vi "Test Search-Split String.vi"(8 "error in (no error)":errorcluster) -> (0 "error out":errorcluster, 3 "Pass?":bool)   [LabVIEW 2020]
uses:
  G-Unicode/Types/UTF-8 String/UTF-8 String.lvclass/UTF-8 String.ctl
  9ff3dfa9-f8ba-4427-ad5f-a2fde7b6c77a.vi
  850149eb-9a48-45f9-aca9-3728815fdd3d.vi
  d33158b6-7e12-4a86-8fbe-645f2238ccec.vi
  2fcd0a92-766f-4ab9-bfdc-e2927028f498.vi
  451e0aa1-621d-4b4c-868c-abfc6350e238.vi
  77c8659a-ed0f-4c8d-a4b1-7b3f6f0d4640.vi
  G-Unicode/Private/Conversion/String as Encoded String.vi
  G-Unicode/Private/Conversion/Polymorphic VIs/String as Encoded String (LabVIEW String).vi
  G-Unicode/Private/Library/gu_search_split_string.vi
  850149eb-9a48-45f9-aca9-3728815fdd3d.vi/3a31b270-3bb6-4c58-a256-c5fcc2c98f09.vi
  850149eb-9a48-45f9-aca9-3728815fdd3d.vi/0ec5df2d-ef9b-4f84-a6a8-ffcedd45c4dc.vi
  d33158b6-7e12-4a86-8fbe-645f2238ccec.vi/3a31b270-3bb6-4c58-a256-c5fcc2c98f09.vi
  d33158b6-7e12-4a86-8fbe-645f2238ccec.vi/0ec5df2d-ef9b-4f84-a6a8-ffcedd45c4dc.vi
  451e0aa1-621d-4b4c-868c-abfc6350e238.vi/3a31b270-3bb6-4c58-a256-c5fcc2c98f09.vi
  451e0aa1-621d-4b4c-868c-abfc6350e238.vi/0ec5df2d-ef9b-4f84-a6a8-ffcedd45c4dc.vi
  77c8659a-ed0f-4c8d-a4b1-7b3f6f0d4640.vi/3a31b270-3bb6-4c58-a256-c5fcc2c98f09.vi
  77c8659a-ed0f-4c8d-a4b1-7b3f6f0d4640.vi/0ec5df2d-ef9b-4f84-a6a8-ffcedd45c4dc.vi
  G-Unicode/Private/Conversion/Text to UTF-8.vi
  G-Unicode/Private/Conversion/Polymorphic VIs/Text to UTF-8 (LabVIEW String).vi
  G-Unicode/Private/Memory/Copy String.vi
  G-Unicode/Private/Library/Result To Error.vi
  G-Unicode/Private/Conversion/Text as Encoded String.vi
  G-Unicode/Private/Conversion/Polymorphic VIs/Text as Encoded String (LabVIEW String).vi
  G-Unicode/Private/Conversion/Polymorphic VIs/Text as Encoded String (UTF-8 String).vi
  G-Unicode/Private/Memory/Copy String.vi/4d47babd-4a2d-4eb7-b91b-7e707d692665.vi
  G-Unicode/Private/Library/gu_free.vi
  G-Unicode/Types/UTF-8 String/Read Encoded UTF-8 String.vi
  <vilib>/Utility/error.llb/Error Cluster From Error Code.vi
  G-Unicode/Types/UTF-8 String/UTF-8 String.lvclass
  f040e557-eb9e-442d-a968-7fe909837c60.vi
  G-Unicode/Unicode/Controls/String Encoding.ctl
  G-Unicode/G-Unicode.lvlib
  6d55fd50-21d3-485a-937b-971210f7077f.vi
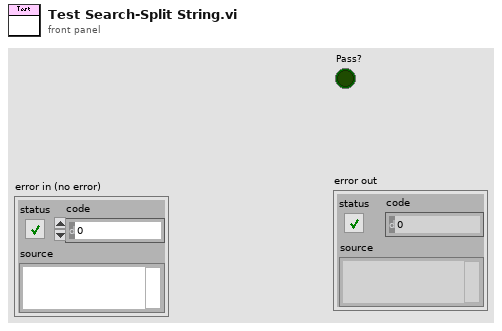
[diagram p1: front panel]
types:
  T1 = typedef "G-Unicode.lvlib/String Encoding.ctl" = enum16{"ANSI", "UTF-8", "UTF-16LE", "UTF-16BE", "Unknown"}
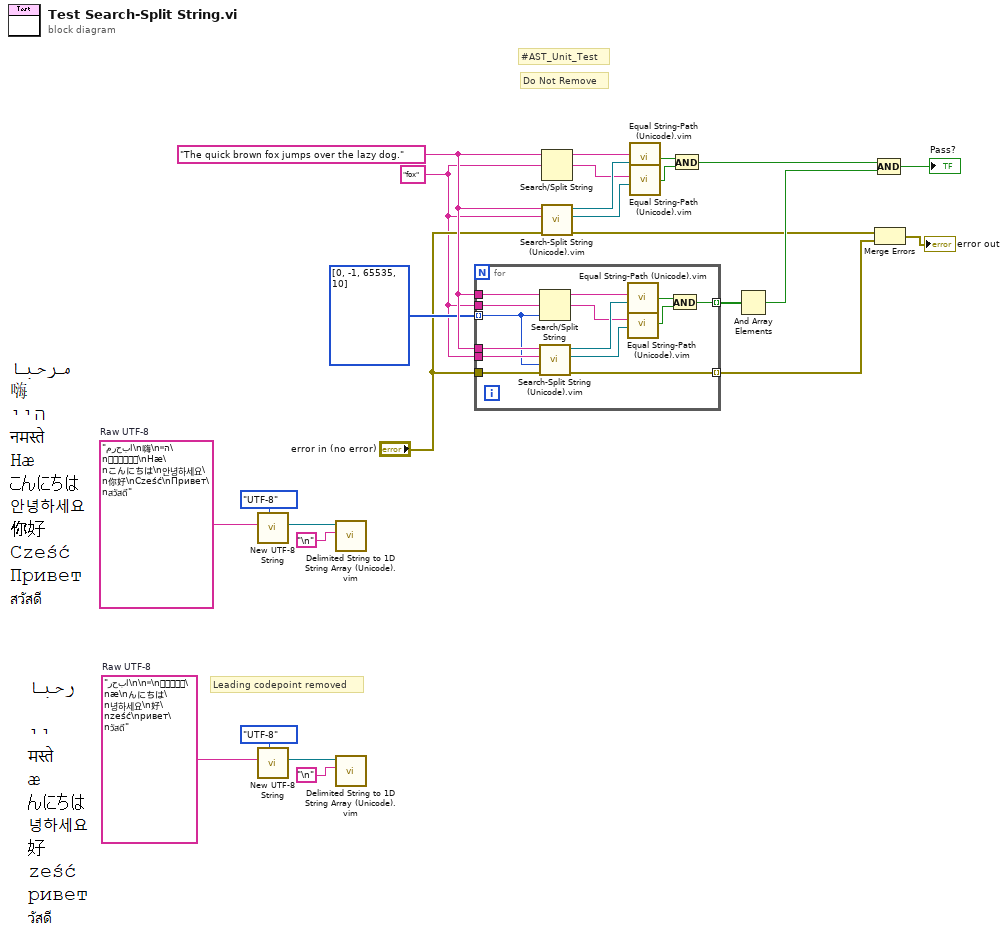
[diagram p0: block diagram]
diagram:
  w9 = "fox" ("search string/char (-)")
  w1 = "رحبا\n\nיי\nमस्ते\næ\nんにちは\n녕하세요\n好\nześć\nривет\nวัสดี"  # Raw UTF-8
  w18 = "The quick brown fox jumps over the lazy dog." ("string")
  w2 = "مرحبا\n嗨\nהיי\nनमस्ते\nHæ\nこんにちは\n안녕하세요\n你好\nCześć\nПривет\nสวัสดี"  # Raw UTF-8
  # "Leading codepoint removed"
  # "Do Not Remove"
  # "#AST_Unit_Test"
  n1 = call "New UTF-8 String.vi"("Input Encoding (ANSI)"=String_Encoding."UTF-8", "String"=w2) -> ("UTF-8 String"=w7:refnum<class "UTF-8 String.lvclass">)  [unwired: 8 in, 1 out]
  n2 = call "New UTF-8 String.vi"("Input Encoding (ANSI)"=String_Encoding."UTF-8", "String"=w1) -> ("UTF-8 String"=w4:refnum<class "UTF-8 String.lvclass">)  [unwired: 8 in, 1 out]
  n3 = call "Delimited String to 1D String Array (Unicode).vim"("Delimiter (tab)"="\n", "Delimited String"=w7) -> ()  [unwired: 8 in, 2 out]
  n4 = call "Delimited String to 1D String Array (Unicode).vim"("Delimiter (tab)"="\n", "Delimited String"=w4) -> ()  [unwired: 8 in, 2 out]
  n5 = for {
    tunnel: [w35] -> w16 mode=indexing
    tunnel: w18 -> [w34]
    tunnel: w9 -> [w33]
    tunnel: w18 -> [w32]
    tunnel: w9 -> [w31]
    tunnel: "error in (no error)" -> [w30]
    tunnel: [w28] -> w17 mode=indexing
    tunnel: i32[] [0, -1, 65535, 10] -> [w26] mode=indexing
    n6 = Search/Split String(string=w34, search string/char (-)=w33, offset (0)=w26) -> (substring before match=w29:string, match + rest of string=w27:string)  [unwired: 1 out]
    n7 = call "Search-Split String (Unicode).vim"("error in"=w30, "Offset (0)"=w26, "Search String/Codepoint"=w31, "String"=w32) -> ("error out"=w28:errorcluster, "Match + Rest Of String"=w37:refnum<class "UTF-8 String.lvclass">, "Substring Before Match"=w36:refnum<class "UTF-8 String.lvclass">)  [unwired: 5 in]
    n8 = call "Equal String-Path (Unicode).vim"("y"=w36, "x"=w29) -> ("Equal?"=w38:bool)  [unwired: 7 in, 1 out]
    n9 = call "Equal String-Path (Unicode).vim"("y"=w37, "x"=w27) -> ("Equal?"=w39:bool)  [unwired: 7 in, 1 out]
    n10 = And(x=w38, y=w39) -> (x .and. y?=w35:bool)
  }
  n11 = Search/Split String(string=w18, search string/char (-)=w9) -> (substring before match=w13:string, match + rest of string=w11:string)  [unwired: 1 in, 1 out]
  n12 = call "Search-Split String (Unicode).vim"("error in"="error in (no error)", "Search String/Codepoint"=w9, "String"=w18) -> ("error out"=w12:errorcluster, "Match + Rest Of String"=w22:refnum<class "UTF-8 String.lvclass">, "Substring Before Match"=w24:refnum<class "UTF-8 String.lvclass">)  [unwired: 6 in]
  n13 = call "Equal String-Path (Unicode).vim"("y"=w24, "x"=w13) -> ("Equal?"=w21:bool)  [unwired: 7 in, 1 out]
  n14 = call "Equal String-Path (Unicode).vim"("y"=w22, "x"=w11) -> ("Equal?"=w20:bool)  [unwired: 7 in, 1 out]
  n15 = And(x=w21, y=w20) -> (x .and. y?=w19:bool)
  n16 = And Array Elements(Boolean array=w16) -> (logical AND=w15:bool)
  n17 = Merge Errors(w12, w17) -> (→"error out":errorcluster)
  n18 = Compound Arithmetic op=AND(w19, w15) -> (→"Pass?":bool)
